vi "GDSLvIcon_GenerateObjectIcon.vi"(1 "HeaderColor":u32(colorbox)=786176, 3 "BackgroundColor":u32(colorbox)=16775072, 4 "Height":u32=22, 5 "error in (no error)":errorcluster, 6 "Type":T1, 7 "Width(30)":u32=30, 8 "ClassBodyIcon":string, 9 "_Thickness":u8=1 caption="Thickness (pixels)" min=1 max=3 step=1) -> (15 "BodyIconOut":u8[][](array[numeric])=[[2, 2, 2, 2, 2, 2, 2, 2, 2, 2, 2, 2, 2, 2, 2, 2, 2, 2, 2, 2, 2, 2, 2, 2, 2, 2, 2, 2, 2, 2], [2, 2, 2, 2, 2, 2, 2, 2, 2, 2, 2, 2, 2, 2, 185, 185, 2, 2, 2, 2, 2, 2, 2, 2, 2, 2, 2, 2, 2, 2], [2, 2, 2, 2, 2, 2, 2, 2, 2, 2, 2, 2, 185, 229, 227, 229, 229, 185, 2, 2, 2, 2, 2, 2, 2, 2, 2, 2, 2, 2], [2, 2, 2, 2, 2, 2, 2, 2, 2, 2, 185, 229, 227, 185, 185, 185, 185, 229, 229, 185, 2, 2, 2, 2, 2, 2, 2, 2, 2, 2], [2, 2, 2, 2, 2, 2, 2, 2, 185, 229, 227, 185, 185, 185, 185, 185, 185, 185, 185, 229, 229, 185, 2, 2, 2, 2, 2, 2, 2, 2], [2, 2, 2, 2, 2, 2, 2, 229, 227, 185, 185, 185, 185, 185, 185, 185, 185, 185, 185, 185, 185, 229, 229, 2, 2, 2, 2, 2, 2, 2], [2, 2, 2, 2, 2, 2, 2, 227, 227, 185, 185, 185, 185, 185, 185, 185, 185, 185, 185, 185, 185, 232, 229, 2, 2, 2, 2, 2, 2, 2], [2, 2, 2, 2, 2, 2, 2, 227, 229, 229, 227, 185, 185, 185, 185, 185, 185, 185, 185, 232, 232, 232, 227, 2, 2, 2, 2, 2, 2, 2], [2, 2, 2, 2, 2, 2, 2, 227, 229, 229, 229, 229, 227, 185, 185, 185, 185, 232, 232, 232, 232, 232, 227, 2, 2, 2, 2, 2, 2, 2], [2, 2, 2, 2, 2, 2, 2, 227, 229, 229, 229, 229, 229, 229, 227, 229, 232, 232, 232, 232, 232, 232, 227, 2, 2, 2, 2, 2, 2, 2], [2, 2, 2, 2, 2, 2, 2, 227, 229, 229, 229, 229, 229, 229, 229, 232, 232, 232, 232, 232, 232, 232, 227, 2, 2, 2, 2, 2, 2, 2], [2, 2, 2, 2, 2, 2, 2, 227, 229, 229, 229, 229, 229, 229, 229, 232, 232, 232, 232, 232, 232, 232, 227, 2, 2, 2, 2, 2, 2, 2], [2, 2, 2, 2, 2, 2, 2, 227, 229, 229, 229, 229, 229, 229, 229, 232, 232, 232, 232, 232, 232, 232, 227, 2, 2, 2, 2, 2, 2, 2], [2, 2, 2, 2, 2, 2, 2, 227, 229, 229, 229, 229, 229, 229, 229, 232, 232, 232, 232, 232, 232, 232, 227, 2, 2, 2, 2, 2, 2, 2], [2, 2, 2, 2, 2, 2, 2, 227, 229, 229, 229, 229, 229, 229, 229, 232, 232, 232, 232, 232, 232, 232, 227, 2, 2, 2, 2, 2, 2, 2], [2, 2, 2, 2, 2, 2, 2, 229, 229, 229, 229, 229, 229, 229, 229, 232, 232, 232, 232, 232, 232, 229, 229, 172, 172, 172, 2, 2, 2, 2], [2, 2, 2, 2, 2, 2, 2, 2, 227, 227, 229, 229, 229, 229, 229, 232, 232, 232, 232, 229, 229, 227, 172, 172, 172, 172, 172, 172, 2, 2], [2, 2, 2, 2, 2, 2, 2, 2, 2, 2, 227, 229, 229, 229, 229, 232, 232, 229, 229, 227, 172, 172, 172, 172, 172, 172, 2, 2, 2, 2], [2, 2, 2, 2, 2, 2, 2, 2, 2, 2, 2, 2, 227, 229, 229, 229, 229, 185, 172, 172, 172, 172, 172, 172, 172, 2, 2, 2, 2, 2], [2, 2, 2, 2, 2, 2, 2, 2, 2, 2, 2, 2, 2, 2, 227, 185, 172, 172, 172, 172, 172, 172, 172, 2, 2, 2, 2, 2, 2, 2], [2, 2, 2, 2, 2, 2, 2, 2, 2, 2, 2, 2, 2, 2, 2, 2, 2, 172, 172, 172, 172, 2, 2, 2, 2, 2, 2, 2, 2, 2], [2, 2, 2, 2, 2, 2, 2, 2, 2, 2, 2, 2, 2, 2, 2, 2, 2, 2, 2, 2, 2, 2, 2, 2, 2, 2, 2, 2, 2, 2]] format="%x", 19 "error out":errorcluster)   [LabVIEW 2020]
uses:
  <resource>/Framework/Providers/Open_GDS/ClassProviders/Common/LvIcon_class/GDSLvIcon_Type.ctl
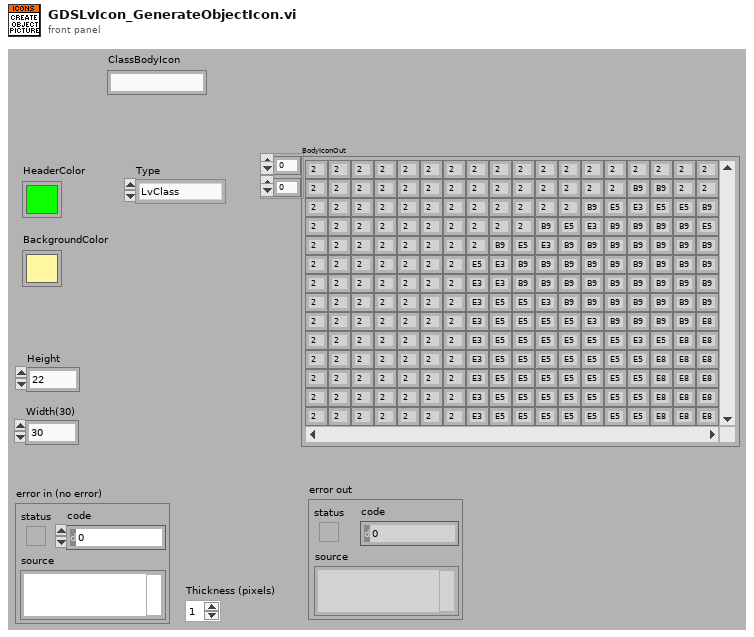
[diagram p1: front panel]
types:
  T1 = typedef "GDSLvIcon_Type.ctl" = enum16{"LvClass", "Library", "X-Control", "LvInterface"}
  T2 = typedef "imagedata.ctl" = cluster{"image type":i32, "image depth":i32, "image":u8[], "mask":u8[], "colors":u32[], "Rectangle":cluster{"left":i16, "top":i16, "right":i16, "bottom":i16}}
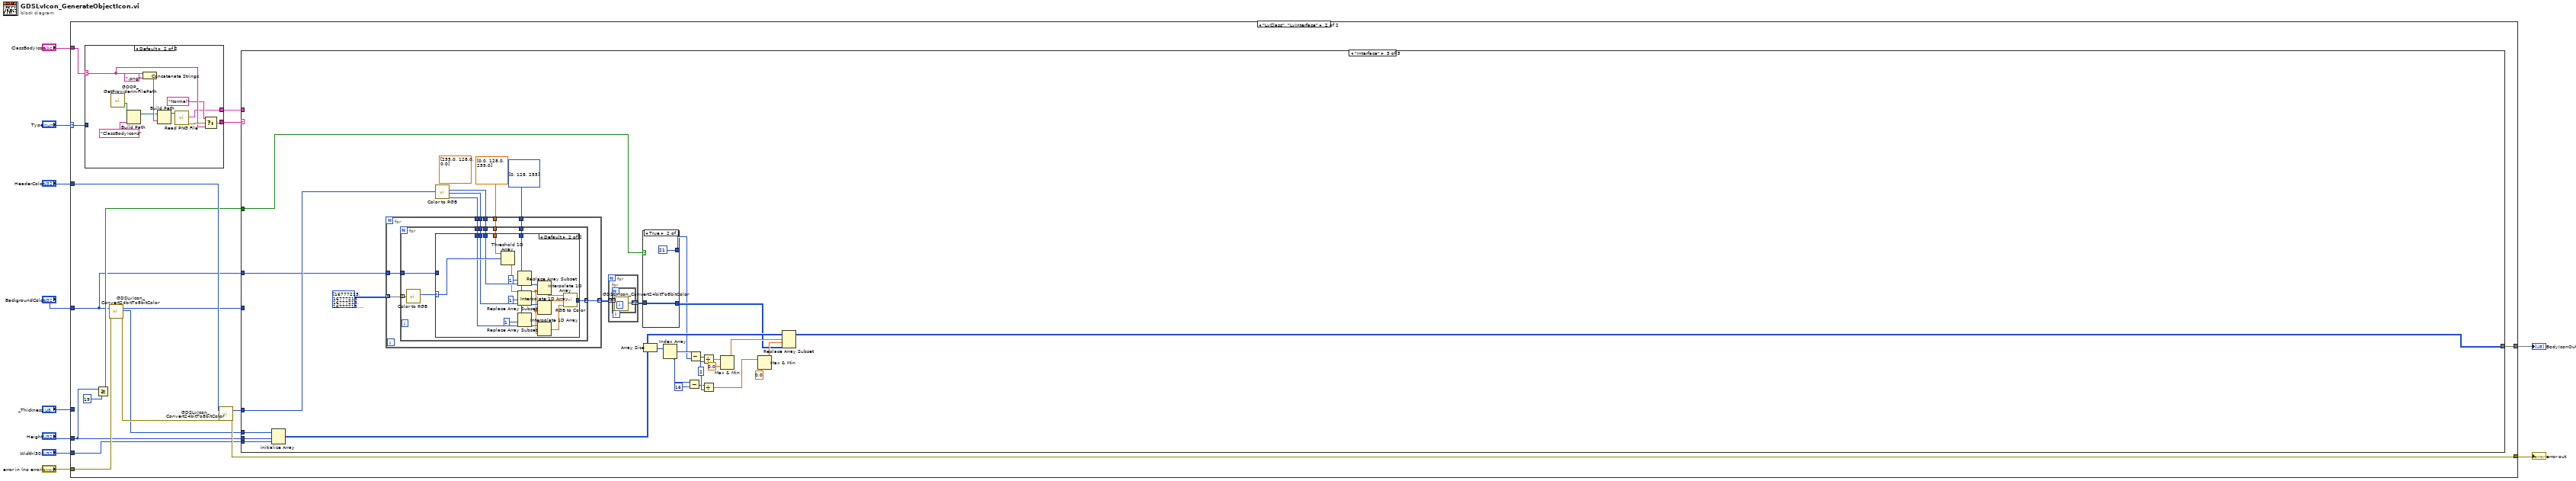
[diagram p0: block diagram]
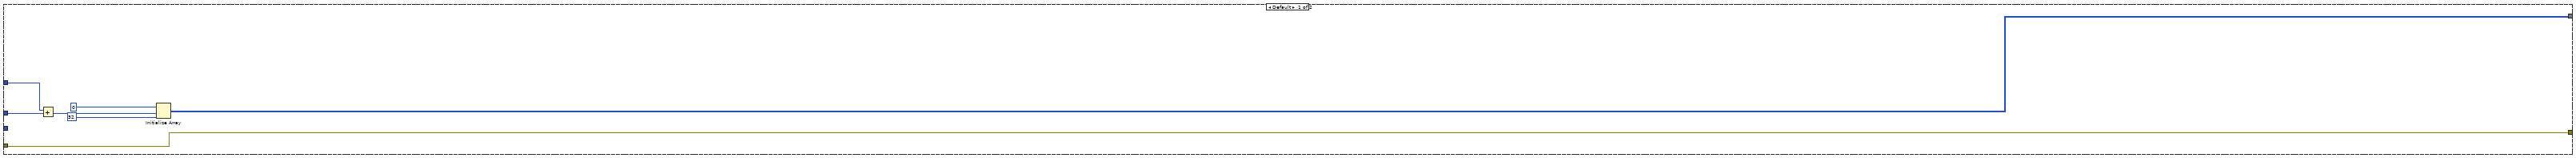
[diagram p2: hidden frame]
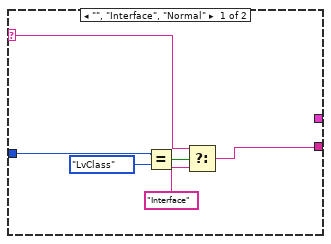
[diagram p3: hidden frame]
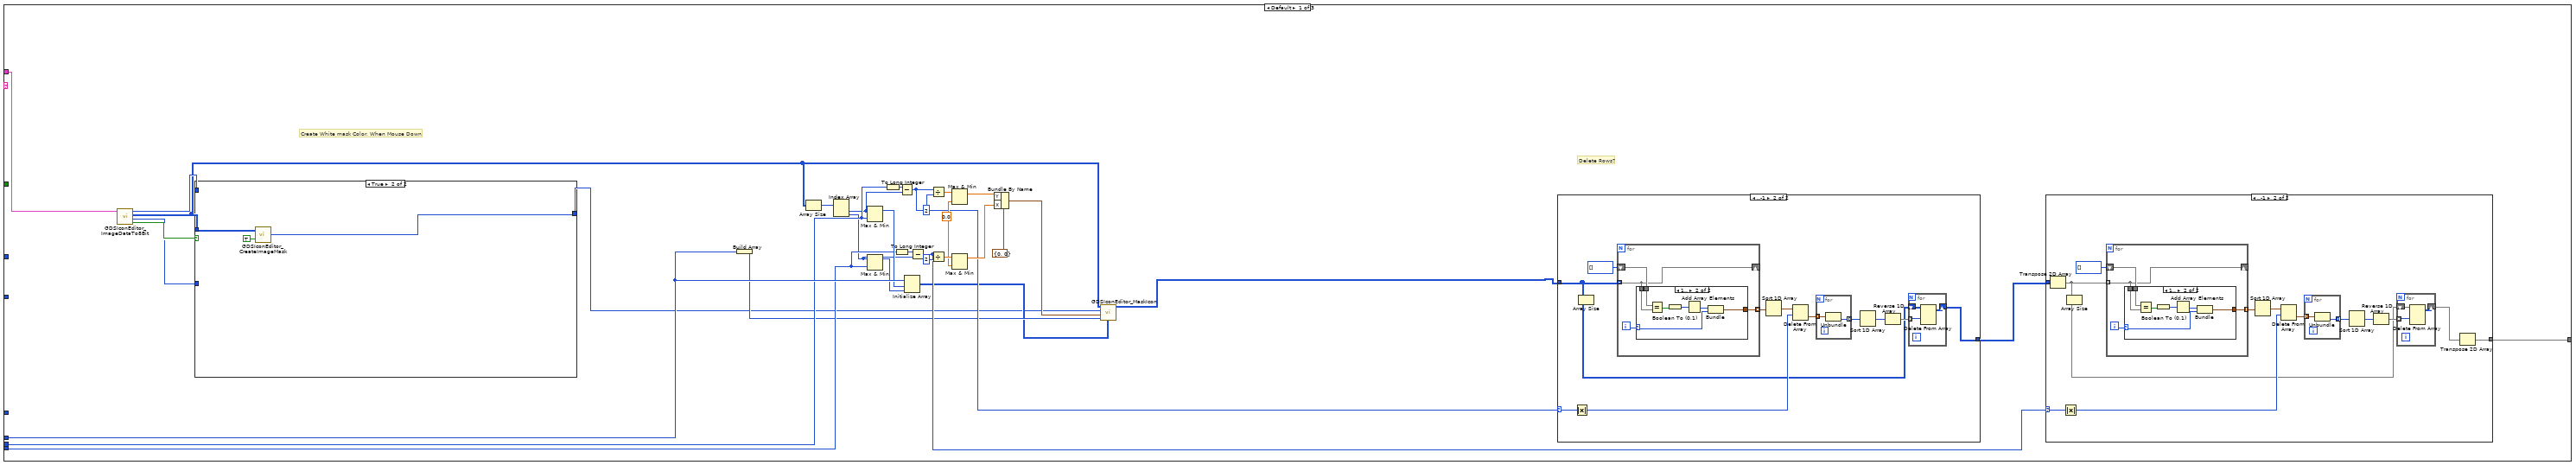
[diagram p4: hidden frame]
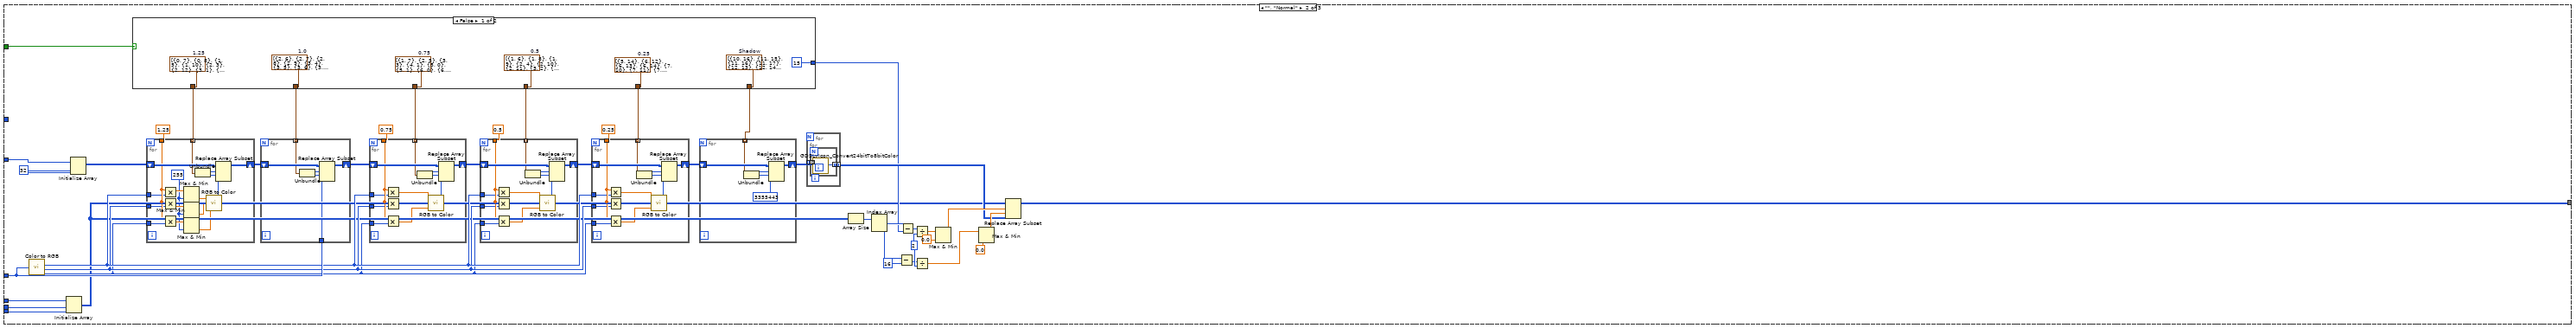
[diagram p10: hidden frame]
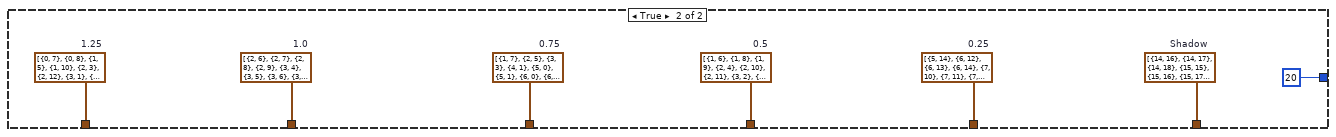
[diagram p11: hidden frame]
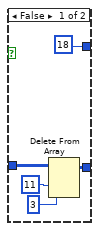
[diagram p12: hidden frame]
diagram:
  n1 = case shown="\"LvClass\", \"LvInterface\"" "Type" {
    selector: "Type" -> [_ w19]
    tunnel: "HeaderColor" -> [_ w34]
    tunnel: [w15 w32] -> w9
    tunnel: "BackgroundColor" -> [_ w18]
    tunnel: "error in (no error)" -> [w15 w31]
    tunnel: "Width(30)" -> [_ w20]
    tunnel: "Height" -> [w13 w21]
    tunnel: [w16 w24] -> w4
    tunnel: "_Thickness" -> [w12 _]
    tunnel: "ClassBodyIcon" -> [_ w26]
    frame Default {
      n2 = Add(x=w12, y=w13) -> (x+y=w11:u32)
      n3 = Initialize Array(u8 0 ("element"), w11, 32 ("dimension size")) -> (w16:u8[][])
    }
    frame "LvClass", "LvInterface" {
      n4 = case shown="Default" w26 {
        selector: w26 -> [w37 w44]
        tunnel: [w36 w43] -> w25
        tunnel: [_ w41] -> w23
        tunnel: w19 -> [w40 _]
        frame "", "Interface", "Normal" {
          n5 = Equal?(x=w40, y=GDSLvIcon_Type."LvClass") -> (x = y?=w38:bool)
          n6 = Select(t=w37, s=w38, f="Interface") -> (s? t:f=w36:string)
        }
        frame Default {
          n7 = call <resource>:"GOOP_GetProviderIniFilePath.vi"() -> ("ProviderMainFolder"=w48:path)  [unwired: 10 in, 1 out]
          n8 = Build Path(base path=w48, name or relative path="ClassBodyIcons") -> (appended path=w50:path)
          n9 = Concatenate Strings(w44, ".png" ("string")) -> (w51:string)
          n10 = Build Path(base path=w50, name or relative path=w51) -> (appended path=w46:path)
          n11 = call <vilib>:"Read PNG File.vi"("path to PNG file"=w46) -> ("error out"=w45:errorcluster, "image data"=w41:T2)  [unwired: 8 in, 1 out]
          n12 = Select(t="Normal", s=w45, f=w44) -> (s? t:f=w43:string)
        }
      }
      n13 = Greater Or Equal?(x=w21, y=19) -> (x >= y?=w28:bool)
      n14 = call <resource>:"GDSLvIcon_Convert24bitTo8bitColor.vi"("Color 24bit In"=w18, "error in (no error)"=w31) -> ("Adjusted 24bit Color Out"=w27:u32, "Color out(256)"=w22:u8, "error out"=w30:errorcluster)  [unwired: 14 in, 1 out]
      n15 = call <resource>:"GDSLvIcon_Convert24bitTo8bitColor.vi"("Color 24bit In"=w34, "error in (no error)"=w30) -> ("Adjusted 24bit Color Out"=w33:u32, "error out"=w32:errorcluster)  [unwired: 14 in, 2 out]
      n16 = case shown="\"Interface\"" w25 {
        tunnel: w33 -> [_ w186 w301]
        tunnel: w28 -> [_ w168 w277]
        tunnel: w27 -> [_ w167 _]
        tunnel: [w59 w150 w283] -> w24
        tunnel: w23 -> [w81 _ _]
        tunnel: w22 -> [w79 w149 w287]
        tunnel: w21 -> [w76 w148 w286]
        tunnel: w20 -> [w68 w147 w285]
        tunnel: w18 -> [_ _ w281]
        frame Default {
          w65 = 0.0 ("y")
          # "Delete Rows?"
          # "Create White mask Color, When Mouse Down"
          n17 = call <resource>:"GDSIconEditor_ImageDataTo8Bit.vi"("image data"=w81) -> ("NoMaskFound"=w83:bool, "ColorArray"=w58:u32[], "8-bit pixmap"=w55:u8[][], "mask"=w82:u8[])  [unwired: 7 in]
          n18 = case shown="True" w83 {
            tunnel: w55 -> [_ w145]
            tunnel: w82 -> [w142 _]
            tunnel: [w142 w143] -> w52
            tunnel: w58 -> [_ _]
            frame False {
            }
            frame True {
              n19 = call <resource>:"GDSIconEditor_CreateImageMask.vi"("Flood Fill"=TRUE, "8-bit pixmap"=w145) -> ("Array"=w143:u8[])
            }
          }
          n20 = Build Array(w79) -> (w56:u8[])
          n21 = Array Size(array=w55) -> (size(s)=w80:i32[])
          n22 = Index Array(array=w80) -> (element #1=w75:i32, element #2=w67:i32)  [unwired: 2 in]
          n23 = Max & Min(x=w75, y=w76) -> (max(x,y)=w78:u32)  [unwired: 1 out]
          n24 = Max & Min(x=w67, y=w68) -> (max(x,y)=w77:u32)  [unwired: 1 out]
          n25 = To Long Integer(number=w76) -> (32bit integer=w64:i32)
          n26 = To Long Integer(number=w68) -> (32bit integer=w63:i32)
          n27 = Subtract(x=w64, y=w75) -> (x-y=w62:i32)
          n28 = Initialize Array(w79, w78, w77) -> (w53:u8[][])
          n29 = Subtract(x=w63, y=w67) -> (x-y=w60:i32)
          n30 = Divide(x=w62, y=u32 2) -> (x/y=w73:dbl)
          n31 = Divide(x=w60, y=u32 2) -> (x/y=w70:dbl)
          n32 = Max & Min(x=w73, y=w65) -> (max(x,y)=w71:dbl)  [unwired: 1 out]
          n33 = Max & Min(x=w70, y=w65) -> (max(x,y)=w66:dbl)  [unwired: 1 out]
          n34 = Bundle By Name(cluster=cluster{"X":i32, "Y":i32} {"X"=0, "Y"=0} ("BgIconOffset"), "Y"=w71, "X"=w66) -> (w57:cluster{"X":i32, "Y":i32})
          n35 = call <resource>:"GDSIconEditor_MaskIcon.vi"("BgIcon"=w53, "ColorsOkayforiconToBeOnTopOf"=w56, "BgIconOffset"=w57, "BgIconMask"=w52, "IconIn"=w55) -> ("IconOut"=w54:u8[][])  [unwired: 6 in]
          n36 = case shown="..-1" w62 {
            selector: w62 -> [_ w125]
            tunnel: w54 -> [w114 w115]
            tunnel: [w114 w116] -> w61
            frame Default {
            }
            frame ..-1 {
              n37 = Absolute Value(x=w125) -> (abs(x)=w121:i32)
              n38 = Array Size(array=w115) -> ()  [unwired: 1 out]
              n39 = for {
                tunnel: w115 -> [w132] mode=indexing
                shift-right: [w132] -> _
                shift-left: u8[] [] -> [w133]
                tunnel: [w131] -> w123 mode=indexing
                i -> [w134]
                n40 = case shown="1.." w134 {
                  selector: w134 -> [_ w136]
                  tunnel: w133 -> [_ w141]
                  tunnel: w132 -> [_ w140]
                  tunnel: [_ w135] -> w131
                  frame 0, Default {
                  }
                  frame 1.. {
                    n41 = Equal?(x=w141, y=w140) -> (x = y?=w139:bool[])
                    n42 = Boolean To (0,1)(Boolean=w139) -> (0, 1=w138:i16[])
                    n43 = Add Array Elements(numeric array=w138) -> (sum=w137:i16)
                    n44 = Bundle("Color out(256)"=w137, w136) -> (w135:cluster{"Color out(256)":i16, i32})  [unwired: 1 in]
                  }
                }
              }
              n45 = Sort 1D Array(array=w123) -> (sorted array=w122:cluster{"Color out(256)":i16, i32}[])
              n46 = Delete From Array(array=w122, length=w121) -> (deleted portion=w120:cluster{"Color out(256)":i16, i32}[])  [unwired: 1 in, 1 out]
              n47 = for {
                tunnel: w120 -> [w130] mode=indexing
                tunnel: [w129] -> w119 mode=indexing
                n48 = Unbundle(w130) -> (w129:i32)  [unwired: 1 out]
              }
              n49 = Sort 1D Array(array=w119) -> (sorted array=w118:i32[])
              n50 = Reverse 1D Array(array=w118) -> (reversed array=w117:i32[])
              n51 = for {
                tunnel: w117 -> [w126] mode=indexing
                shift-right: [w127] -> w116
                shift-left: w115 -> [w128]
                n52 = Delete From Array(array=w128, index (row)=w126) -> (array with subset deleted=w127:u8[][])  [unwired: 2 in, 1 out]
              }
            }
          }
          n53 = case shown="..-1" w60 {
            selector: w60 -> [_ w97]
            tunnel: w61 -> [w84 w87]
            tunnel: [w84 w85] -> w59
            frame Default {
            }
            frame ..-1 {
              n54 = Transpose 2D Array(2D array=w87) -> (transposed array=w86:u8[][])
              n55 = Absolute Value(x=w97) -> (abs(x)=w93:i32)
              n56 = Array Size(array=w86) -> ()  [unwired: 1 out]
              n57 = for {
                tunnel: w86 -> [w104] mode=indexing
                shift-right: [w104] -> _
                shift-left: u8[] [] -> [w105]
                tunnel: [w103] -> w95 mode=indexing
                i -> [w106]
                n58 = case shown="1.." w106 {
                  selector: w106 -> [_ w108]
                  tunnel: w105 -> [_ w113]
                  tunnel: w104 -> [_ w112]
                  tunnel: [_ w107] -> w103
                  frame 0, Default {
                  }
                  frame 1.. {
                    n59 = Equal?(x=w113, y=w112) -> (x = y?=w111:bool[])
                    n60 = Boolean To (0,1)(Boolean=w111) -> (0, 1=w110:i16[])
                    n61 = Add Array Elements(numeric array=w110) -> (sum=w109:i16)
                    n62 = Bundle("Color out(256)"=w109, w108) -> (w107:cluster{"Color out(256)":i16, i32})  [unwired: 1 in]
                  }
                }
              }
              n63 = Sort 1D Array(array=w95) -> (sorted array=w94:cluster{"Color out(256)":i16, i32}[])
              n64 = Delete From Array(array=w94, length=w93) -> (deleted portion=w92:cluster{"Color out(256)":i16, i32}[])  [unwired: 1 in, 1 out]
              n65 = for {
                tunnel: w92 -> [w102] mode=indexing
                tunnel: [w101] -> w91 mode=indexing
                n66 = Unbundle(w102) -> (w101:i32)  [unwired: 1 out]
              }
              n67 = Sort 1D Array(array=w91) -> (sorted array=w90:i32[])
              n68 = Reverse 1D Array(array=w90) -> (reversed array=w89:i32[])
              n69 = for {
                tunnel: w89 -> [w98] mode=indexing
                shift-right: [w99] -> w88
                shift-left: w86 -> [w100]
                n70 = Delete From Array(array=w100, index (row)=w98) -> (array with subset deleted=w99:u8[][])  [unwired: 2 in, 1 out]
              }
              n71 = Transpose 2D Array(2D array=w88) -> (transposed array=w85:u8[][])
            }
          }
        }
        frame "", "Normal" {
          w157 = 2 ("y")
          w175 = 32 ("dimension size")
          n72 = call <vilib>:"Color to RGB.vi"("Color"=w186) -> ("R"=w178:u8, "G"=w177:u8, "B"=w176:u8)  [unwired: 1 out]
          n73 = Initialize Array(w149, w148, w147) -> (w146:u8[][])
          n74 = Initialize Array(w167, w175, w175) -> (w189:u32[][])
          n75 = case shown="False" w168 {
            tunnel: [w195 w207] -> w174
            tunnel: [w196 w206] -> w173
            tunnel: [w197 w205] -> w172
            tunnel: [w198 w204] -> w171
            tunnel: [w199 w203] -> w170
            tunnel: [w200 w202] -> w169
            tunnel: [15 ("y") 20 ("y")] -> w151
            frame False {
              w195 = cluster{"X":i32, "Y":i32}[] [{"X"=0, "Y"=7}, {"X"=0, "Y"=8}, {"X"=1, "Y"=5}, {"X"=1, "Y"=10}, {"X"=2, "Y"=3}, {"X"=2, "Y"=12}, {"X"=3, "Y"=1}, {"X"=3, "Y"=14}]  # 1.25
              w196 = cluster{"X":i32, "Y":i32}[] [{"X"=2, "Y"=6}, {"X"=2, "Y"=7}, {"X"=2, "Y"=8}, {"X"=2, "Y"=9}, {"X"=3, "Y"=4}, {"X"=3, "Y"=5}, {"X"=3, "Y"=6}, {"X"=3, "Y"=7}, {"X"=3, "Y"=8}, {"X"=3, "Y"=9}, {"X"=3, "Y"=10}, {"X"=3, "Y"=11}, {"X"=4, "Y"=2}, {"X"=4, "Y"=3}, {"X"=4, "Y"=4}, {"X"=4, "Y"=5}, {"X"=4, "Y"=6}, {"X"=4, "Y"=7}, {"X"=4, "Y"=8}, {"X"=4, "Y"=9}, {"X"=4, "Y"=10}, {"X"=4, "Y"=11}, {"X"=4, "Y"=12}, {"X"=4, "Y"=13}, {"X"=5, "Y"=2}, {"X"=5, "Y"=3}, {"X"=5, "Y"=4}, {"X"=5, "Y"=5}, {"X"=5, "Y"=6}, {"X"=5, "Y"=7}, {"X"=5, "Y"=8}, {"X"=5, "Y"=9}, {"X"=5, "Y"=10}, {"X"=5, "Y"=11}, {"X"=5, "Y"=12}, {"X"=5, "Y"=13}, {"X"=6, "Y"=4}, {"X"=6, "Y"=5}, {"X"=6, "Y"=6}, {"X"=6, "Y"=7}, {"X"=6, "Y"=8}, {"X"=6, "Y"=9}, {"X"=6, "Y"=10}, {"X"=6, "Y"=11}, {"X"=7, "Y"=6}, {"X"=7, "Y"=7}, {"X"=7, "Y"=8}, {"X"=7, "Y"=9}, {"X"=13, "Y"=10}, {"X"=14, "Y"=8}]  # 1.0
              w198 = cluster{"X":i32, "Y":i32}[] [{"X"=1, "Y"=6}, {"X"=1, "Y"=8}, {"X"=1, "Y"=9}, {"X"=2, "Y"=4}, {"X"=2, "Y"=10}, {"X"=2, "Y"=11}, {"X"=3, "Y"=2}, {"X"=3, "Y"=12}, {"X"=3, "Y"=13}, {"X"=4, "Y"=0}, {"X"=4, "Y"=14}, {"X"=4, "Y"=15}, {"X"=5, "Y"=15}, {"X"=6, "Y"=1}, {"X"=6, "Y"=2}, {"X"=7, "Y"=1}, {"X"=7, "Y"=2}, {"X"=7, "Y"=3}, {"X"=7, "Y"=4}, {"X"=8, "Y"=1}, {"X"=8, "Y"=2}, {"X"=8, "Y"=3}, {"X"=8, "Y"=4}, {"X"=8, "Y"=5}, {"X"=8, "Y"=6}, {"X"=8, "Y"=8}, {"X"=9, "Y"=1}, {"X"=9, "Y"=2}, {"X"=9, "Y"=3}, {"X"=9, "Y"=4}, {"X"=9, "Y"=5}, {"X"=9, "Y"=6}, {"X"=9, "Y"=7}, {"X"=10, "Y"=0}, {"X"=10, "Y"=1}, {"X"=10, "Y"=2}, {"X"=10, "Y"=3}, {"X"=10, "Y"=4}, {"X"=10, "Y"=5}, {"X"=10, "Y"=6}, {"X"=10, "Y"=7}, {"X"=10, "Y"=14}, {"X"=10, "Y"=15}, {"X"=11, "Y"=3}, {"X"=11, "Y"=4}, {"X"=11, "Y"=5}, {"X"=11, "Y"=6}, {"X"=11, "Y"=7}, {"X"=11, "Y"=12}, {"X"=11, "Y"=13}, {"X"=12, "Y"=4}, {"X"=12, "Y"=5}, {"X"=12, "Y"=6}, {"X"=12, "Y"=7}, {"X"=12, "Y"=10}, {"X"=12, "Y"=11}, {"X"=13, "Y"=6}, {"X"=13, "Y"=7}, {"X"=13, "Y"=8}, {"X"=13, "Y"=9}]  # 0.5
              w197 = cluster{"X":i32, "Y":i32}[] [{"X"=1, "Y"=7}, {"X"=2, "Y"=5}, {"X"=3, "Y"=3}, {"X"=4, "Y"=1}, {"X"=5, "Y"=0}, {"X"=5, "Y"=1}, {"X"=6, "Y"=0}, {"X"=6, "Y"=3}, {"X"=6, "Y"=15}, {"X"=7, "Y"=0}, {"X"=7, "Y"=5}, {"X"=7, "Y"=15}, {"X"=8, "Y"=0}, {"X"=8, "Y"=7}, {"X"=8, "Y"=15}, {"X"=9, "Y"=0}, {"X"=9, "Y"=15}, {"X"=11, "Y"=1}, {"X"=11, "Y"=2}, {"X"=11, "Y"=14}, {"X"=12, "Y"=3}, {"X"=12, "Y"=12}, {"X"=13, "Y"=5}, {"X"=14, "Y"=7}]  # 0.75
              w199 = cluster{"X":i32, "Y":i32}[] [{"X"=5, "Y"=14}, {"X"=6, "Y"=12}, {"X"=6, "Y"=13}, {"X"=6, "Y"=14}, {"X"=7, "Y"=10}, {"X"=7, "Y"=11}, {"X"=7, "Y"=12}, {"X"=7, "Y"=13}, {"X"=7, "Y"=14}, {"X"=8, "Y"=9}, {"X"=8, "Y"=10}, {"X"=8, "Y"=11}, {"X"=8, "Y"=12}, {"X"=8, "Y"=13}, {"X"=8, "Y"=14}, {"X"=9, "Y"=8}, {"X"=9, "Y"=9}, {"X"=9, "Y"=10}, {"X"=9, "Y"=11}, {"X"=9, "Y"=12}, {"X"=9, "Y"=13}, {"X"=9, "Y"=14}, {"X"=10, "Y"=8}, {"X"=10, "Y"=9}, {"X"=10, "Y"=10}, {"X"=10, "Y"=11}, {"X"=10, "Y"=12}, {"X"=10, "Y"=13}, {"X"=11, "Y"=8}, {"X"=11, "Y"=9}, {"X"=11, "Y"=10}, {"X"=11, "Y"=11}, {"X"=12, "Y"=8}, {"X"=12, "Y"=9}]  # 0.25
              w200 = cluster{"X":i32, "Y":i32}[] [{"X"=10, "Y"=16}, {"X"=11, "Y"=15}, {"X"=11, "Y"=16}, {"X"=11, "Y"=17}, {"X"=12, "Y"=13}, {"X"=12, "Y"=14}, {"X"=12, "Y"=15}, {"X"=12, "Y"=16}, {"X"=12, "Y"=17}, {"X"=13, "Y"=11}, {"X"=13, "Y"=12}, {"X"=13, "Y"=13}, {"X"=13, "Y"=14}, {"X"=13, "Y"=15}, {"X"=13, "Y"=16}, {"X"=14, "Y"=9}, {"X"=14, "Y"=10}, {"X"=14, "Y"=11}, {"X"=14, "Y"=12}, {"X"=14, "Y"=13}, {"X"=14, "Y"=14}, {"X"=14, "Y"=15}, {"X"=15, "Y"=10}, {"X"=15, "Y"=11}, {"X"=15, "Y"=12}, {"X"=15, "Y"=13}]  # Shadow
            }
            frame True {
              w202 = cluster{"X":i32, "Y":i32}[] [{"X"=14, "Y"=16}, {"X"=14, "Y"=17}, {"X"=14, "Y"=18}, {"X"=15, "Y"=15}, {"X"=15, "Y"=16}, {"X"=15, "Y"=17}, {"X"=15, "Y"=18}, {"X"=15, "Y"=19}, {"X"=15, "Y"=20}, {"X"=16, "Y"=13}, {"X"=16, "Y"=14}, {"X"=16, "Y"=15}, {"X"=16, "Y"=16}, {"X"=16, "Y"=17}, {"X"=16, "Y"=18}, {"X"=17, "Y"=11}, {"X"=17, "Y"=12}, {"X"=17, "Y"=13}, {"X"=17, "Y"=14}, {"X"=17, "Y"=15}, {"X"=17, "Y"=16}, {"X"=17, "Y"=17}, {"X"=18, "Y"=9}, {"X"=18, "Y"=10}, {"X"=18, "Y"=11}, {"X"=18, "Y"=12}, {"X"=18, "Y"=13}, {"X"=18, "Y"=14}, {"X"=18, "Y"=15}, {"X"=19, "Y"=10}, {"X"=19, "Y"=11}, {"X"=19, "Y"=12}, {"X"=19, "Y"=13}]  # Shadow
              w203 = cluster{"X":i32, "Y":i32}[] [{"X"=5, "Y"=14}, {"X"=6, "Y"=12}, {"X"=6, "Y"=13}, {"X"=6, "Y"=14}, {"X"=7, "Y"=10}, {"X"=7, "Y"=11}, {"X"=7, "Y"=12}, {"X"=7, "Y"=13}, {"X"=7, "Y"=14}, {"X"=8, "Y"=9}, {"X"=8, "Y"=10}, {"X"=8, "Y"=11}, {"X"=8, "Y"=12}, {"X"=8, "Y"=13}, {"X"=8, "Y"=14}, {"X"=9, "Y"=8}, {"X"=9, "Y"=9}, {"X"=9, "Y"=10}, {"X"=9, "Y"=11}, {"X"=9, "Y"=12}, {"X"=9, "Y"=13}, {"X"=9, "Y"=14}, {"X"=10, "Y"=8}, {"X"=10, "Y"=9}, {"X"=10, "Y"=10}, {"X"=10, "Y"=11}, {"X"=10, "Y"=12}, {"X"=10, "Y"=13}, {"X"=10, "Y"=14}, {"X"=11, "Y"=8}, {"X"=11, "Y"=9}, {"X"=11, "Y"=10}, {"X"=11, "Y"=11}, {"X"=11, "Y"=12}, {"X"=11, "Y"=13}, {"X"=11, "Y"=14}, {"X"=12, "Y"=8}, {"X"=12, "Y"=9}, {"X"=12, "Y"=10}, {"X"=12, "Y"=11}, {"X"=12, "Y"=12}, {"X"=12, "Y"=13}, {"X"=12, "Y"=14}, {"X"=13, "Y"=8}, {"X"=13, "Y"=9}, {"X"=13, "Y"=10}, {"X"=13, "Y"=11}, {"X"=13, "Y"=12}, {"X"=13, "Y"=13}, {"X"=13, "Y"=14}, {"X"=14, "Y"=8}, {"X"=14, "Y"=9}, {"X"=14, "Y"=10}, {"X"=14, "Y"=11}, {"X"=14, "Y"=12}, {"X"=14, "Y"=13}, {"X"=15, "Y"=8}, {"X"=15, "Y"=9}, {"X"=15, "Y"=10}, {"X"=15, "Y"=11}, {"X"=16, "Y"=8}, {"X"=16, "Y"=9}]  # 0.25
              w205 = cluster{"X":i32, "Y":i32}[] [{"X"=1, "Y"=7}, {"X"=2, "Y"=5}, {"X"=3, "Y"=3}, {"X"=4, "Y"=1}, {"X"=5, "Y"=0}, {"X"=5, "Y"=1}, {"X"=6, "Y"=0}, {"X"=6, "Y"=3}, {"X"=6, "Y"=15}, {"X"=7, "Y"=0}, {"X"=7, "Y"=5}, {"X"=7, "Y"=15}, {"X"=8, "Y"=0}, {"X"=8, "Y"=7}, {"X"=8, "Y"=15}, {"X"=9, "Y"=0}, {"X"=9, "Y"=15}, {"X"=10, "Y"=0}, {"X"=10, "Y"=15}, {"X"=11, "Y"=0}, {"X"=11, "Y"=15}, {"X"=12, "Y"=0}, {"X"=12, "Y"=15}, {"X"=13, "Y"=0}, {"X"=13, "Y"=15}, {"X"=15, "Y"=1}, {"X"=15, "Y"=2}, {"X"=15, "Y"=14}, {"X"=16, "Y"=3}, {"X"=16, "Y"=12}, {"X"=17, "Y"=5}, {"X"=18, "Y"=7}]  # 0.75
              w204 = cluster{"X":i32, "Y":i32}[] [{"X"=1, "Y"=6}, {"X"=1, "Y"=8}, {"X"=1, "Y"=9}, {"X"=2, "Y"=4}, {"X"=2, "Y"=10}, {"X"=2, "Y"=11}, {"X"=3, "Y"=2}, {"X"=3, "Y"=12}, {"X"=3, "Y"=13}, {"X"=4, "Y"=0}, {"X"=4, "Y"=14}, {"X"=4, "Y"=15}, {"X"=5, "Y"=15}, {"X"=6, "Y"=1}, {"X"=6, "Y"=2}, {"X"=7, "Y"=1}, {"X"=7, "Y"=2}, {"X"=7, "Y"=3}, {"X"=7, "Y"=4}, {"X"=8, "Y"=1}, {"X"=8, "Y"=2}, {"X"=8, "Y"=3}, {"X"=8, "Y"=4}, {"X"=8, "Y"=5}, {"X"=8, "Y"=6}, {"X"=8, "Y"=8}, {"X"=9, "Y"=1}, {"X"=9, "Y"=2}, {"X"=9, "Y"=3}, {"X"=9, "Y"=4}, {"X"=9, "Y"=5}, {"X"=9, "Y"=6}, {"X"=9, "Y"=7}, {"X"=10, "Y"=1}, {"X"=10, "Y"=2}, {"X"=10, "Y"=3}, {"X"=10, "Y"=4}, {"X"=10, "Y"=5}, {"X"=10, "Y"=6}, {"X"=10, "Y"=7}, {"X"=11, "Y"=1}, {"X"=11, "Y"=2}, {"X"=11, "Y"=3}, {"X"=11, "Y"=4}, {"X"=11, "Y"=5}, {"X"=11, "Y"=6}, {"X"=11, "Y"=7}, {"X"=12, "Y"=1}, {"X"=12, "Y"=2}, {"X"=12, "Y"=3}, {"X"=12, "Y"=4}, {"X"=12, "Y"=5}, {"X"=12, "Y"=6}, {"X"=12, "Y"=7}, {"X"=13, "Y"=1}, {"X"=13, "Y"=2}, {"X"=13, "Y"=3}, {"X"=13, "Y"=4}, {"X"=13, "Y"=5}, {"X"=13, "Y"=6}, {"X"=13, "Y"=7}, {"X"=14, "Y"=0}, {"X"=14, "Y"=1}, {"X"=14, "Y"=2}, {"X"=14, "Y"=3}, {"X"=14, "Y"=4}, {"X"=14, "Y"=5}, {"X"=14, "Y"=6}, {"X"=14, "Y"=7}, {"X"=14, "Y"=14}, {"X"=14, "Y"=15}, {"X"=15, "Y"=3}, {"X"=15, "Y"=4}, {"X"=15, "Y"=5}, {"X"=15, "Y"=6}, {"X"=15, "Y"=7}, {"X"=15, "Y"=12}, {"X"=15, "Y"=13}, {"X"=16, "Y"=4}, {"X"=16, "Y"=5}, {"X"=16, "Y"=6}, {"X"=16, "Y"=7}, {"X"=16, "Y"=10}, {"X"=16, "Y"=11}, {"X"=17, "Y"=6}, {"X"=17, "Y"=7}, {"X"=17, "Y"=8}, {"X"=17, "Y"=9}]  # 0.5
              w206 = cluster{"X":i32, "Y":i32}[] [{"X"=2, "Y"=6}, {"X"=2, "Y"=7}, {"X"=2, "Y"=8}, {"X"=2, "Y"=9}, {"X"=3, "Y"=4}, {"X"=3, "Y"=5}, {"X"=3, "Y"=6}, {"X"=3, "Y"=7}, {"X"=3, "Y"=8}, {"X"=3, "Y"=9}, {"X"=3, "Y"=10}, {"X"=3, "Y"=11}, {"X"=4, "Y"=2}, {"X"=4, "Y"=3}, {"X"=4, "Y"=4}, {"X"=4, "Y"=5}, {"X"=4, "Y"=6}, {"X"=4, "Y"=7}, {"X"=4, "Y"=8}, {"X"=4, "Y"=9}, {"X"=4, "Y"=10}, {"X"=4, "Y"=11}, {"X"=4, "Y"=12}, {"X"=4, "Y"=13}, {"X"=5, "Y"=2}, {"X"=5, "Y"=3}, {"X"=5, "Y"=4}, {"X"=5, "Y"=5}, {"X"=5, "Y"=6}, {"X"=5, "Y"=7}, {"X"=5, "Y"=8}, {"X"=5, "Y"=9}, {"X"=5, "Y"=10}, {"X"=5, "Y"=11}, {"X"=5, "Y"=12}, {"X"=5, "Y"=13}, {"X"=6, "Y"=4}, {"X"=6, "Y"=5}, {"X"=6, "Y"=6}, {"X"=6, "Y"=7}, {"X"=6, "Y"=8}, {"X"=6, "Y"=9}, {"X"=6, "Y"=10}, {"X"=6, "Y"=11}, {"X"=7, "Y"=6}, {"X"=7, "Y"=7}, {"X"=7, "Y"=8}, {"X"=7, "Y"=9}, {"X"=17, "Y"=10}, {"X"=18, "Y"=8}]  # 1.0
              w207 = cluster{"X":i32, "Y":i32}[] [{"X"=0, "Y"=7}, {"X"=0, "Y"=8}, {"X"=1, "Y"=5}, {"X"=1, "Y"=10}, {"X"=2, "Y"=3}, {"X"=2, "Y"=12}, {"X"=3, "Y"=1}, {"X"=3, "Y"=14}]  # 1.25
            }
          }
          n76 = for {
            shift-right: [w274] -> w187
            shift-left: w189 -> [w275]
            tunnel: w174 -> [w260] mode=indexing
            tunnel: 1.25 ("upper limit") -> [w266]
            tunnel: w178 -> [w265]
            tunnel: w177 -> [w264]
            tunnel: w176 -> [w263]
            w267 = 255 ("upper limit")
            n77 = Multiply(x=w266, y=w265) -> (x*y=w273:dbl)
            n78 = Multiply(x=w266, y=w264) -> (x*y=w269:dbl)
            n79 = Multiply(x=w266, y=w263) -> (x*y=w268:dbl)
            n80 = Max & Min(x=w273, y=w267) -> (min(x,y)=w272:dbl)  [unwired: 1 out]
            n81 = Max & Min(x=w269, y=w267) -> (min(x,y)=w271:dbl)  [unwired: 1 out]
            n82 = Max & Min(x=w268, y=w267) -> (min(x,y)=w270:dbl)  [unwired: 1 out]
            n83 = Unbundle(w260) -> ("X"=w261:i32, "Y"=w259:i32)
            n84 = call <vilib>:"RGB to Color.vi"("B"=w270, "G"=w271, "R"=w272) -> ("Color"=w262:u32)
            n85 = Replace Array Subset(array=w275, new element=w262, index (row)=w261, index (col)=w259) -> (w274:u32[][])
          }
          n86 = for {
            shift-right: [w257] -> w184
            shift-left: w187 -> [w258]
            tunnel: w173 -> [w256] mode=indexing
            tunnel: w186 -> [w255]
            n87 = Unbundle(w256) -> ("X"=w254:i32, "Y"=w253:i32)
            n88 = Replace Array Subset(array=w258, new element=w255, index (row)=w254, index (col)=w253) -> (w257:u32[][])
          }
          n89 = for {
            shift-right: [w251] -> w182
            shift-left: w184 -> [w252]
            tunnel: w172 -> [w250] mode=indexing
            tunnel: 0.75 ("upper limit") -> [w249]
            tunnel: w178 -> [w248]
            tunnel: w177 -> [w247]
            tunnel: w176 -> [w246]
            n90 = Multiply(x=w249, y=w248) -> (x*y=w244:dbl)
            n91 = Multiply(x=w249, y=w247) -> (x*y=w243:dbl)
            n92 = Multiply(x=w249, y=w246) -> (x*y=w242:dbl)
            n93 = Unbundle(w250) -> ("X"=w241:i32, "Y"=w240:i32)
            n94 = call <vilib>:"RGB to Color.vi"("B"=w242, "G"=w243, "R"=w244) -> ("Color"=w245:u32)
            n95 = Replace Array Subset(array=w252, new element=w245, index (row)=w241, index (col)=w240) -> (w251:u32[][])
          }
          n96 = for {
            shift-right: [w238] -> w180
            shift-left: w182 -> [w239]
            tunnel: w171 -> [w237] mode=indexing
            tunnel: 0.5 ("upper limit") -> [w236]
            tunnel: w178 -> [w235]
            tunnel: w177 -> [w234]
            tunnel: w176 -> [w233]
            n97 = Multiply(x=w236, y=w235) -> (x*y=w231:dbl)
            n98 = Multiply(x=w236, y=w234) -> (x*y=w230:dbl)
            n99 = Multiply(x=w236, y=w233) -> (x*y=w229:dbl)
            n100 = Unbundle(w237) -> ("X"=w228:i32, "Y"=w227:i32)
            n101 = call <vilib>:"RGB to Color.vi"("B"=w229, "G"=w230, "R"=w231) -> ("Color"=w232:u32)
            n102 = Replace Array Subset(array=w239, new element=w232, index (row)=w228, index (col)=w227) -> (w238:u32[][])
          }
          n103 = for {
            shift-right: [w225] -> w179
            shift-left: w180 -> [w226]
            tunnel: w170 -> [w224] mode=indexing
            tunnel: 0.25 ("upper limit") -> [w223]
            tunnel: w178 -> [w222]
            tunnel: w177 -> [w221]
            tunnel: w176 -> [w220]
            n104 = Multiply(x=w223, y=w222) -> (x*y=w218:dbl)
            n105 = Multiply(x=w223, y=w221) -> (x*y=w217:dbl)
            n106 = Multiply(x=w223, y=w220) -> (x*y=w216:dbl)
            n107 = Unbundle(w224) -> ("X"=w215:i32, "Y"=w214:i32)
            n108 = call <vilib>:"RGB to Color.vi"("B"=w216, "G"=w217, "R"=w218) -> ("Color"=w219:u32)
            n109 = Replace Array Subset(array=w226, new element=w219, index (row)=w215, index (col)=w214) -> (w225:u32[][])
          }
          n110 = for {
            shift-right: [w212] -> w166
            shift-left: w179 -> [w213]
            tunnel: w169 -> [w211] mode=indexing
            n111 = Unbundle(w211) -> ("X"=w209:i32, "Y"=w208:i32)
            n112 = Replace Array Subset(array=w213, new element=u32 3355443 ("new element/subarray"), index (row)=w209, index (col)=w208) -> (w212:u32[][])
          }
          n113 = for {
            tunnel: w166 -> [w191] mode=indexing
            tunnel: [w190] -> w152 mode=indexing
            n114 = for {
              tunnel: w191 -> [w193] mode=indexing
              tunnel: [w192] -> w190 mode=indexing
              n115 = call <resource>:"GDSLvIcon_Convert24bitTo8bitColor.vi"("Color 24bit In"=w193) -> ("Color out(256)"=w192:u8)  [unwired: 15 in, 3 out]
            }
          }
          n116 = Array Size(array=w146) -> (size(s)=w153:i32[])
          n117 = Index Array(array=w153) -> (element #1=w154:i32, element #2=w158:i32)  [unwired: 2 in]
          n118 = Subtract(x=w158, y=16) -> (x-y=w156:i32)
          n119 = Subtract(x=w154, y=w151) -> (x-y=w155:i32)
          n120 = Divide(x=w155, y=w157) -> (x/y=w161:dbl)
          n121 = Divide(x=w156, y=w157) -> (x/y=w164:dbl)
          n122 = Max & Min(x=w161, y=0.0) -> (max(x,y)=w162:dbl)  [unwired: 1 out]
          n123 = Max & Min(x=w164, y=0.0) -> (max(x,y)=w165:dbl)  [unwired: 1 out]
          n124 = Replace Array Subset(array=w146, new element=w152, index (row)=w162, index (col)=w165) -> (w150:u8[][])
        }
        frame "Interface" {
          w292 = 2 ("y")
          (unwired) sgl[] [255.0, 128.0, 0.0]
          n125 = Initialize Array(w287, w286, w285) -> (w284:u8[][])
          n126 = call <vilib>:"Color to RGB.vi"("Color"=w301) -> ("R"=w304:u8, "G"=w305:u8, "B"=w306:u8)  [unwired: 1 out]
          n127 = for {
            tunnel: u32[][] [[16777215, 16777215, 16777215, 16777215, 16777215, 16777215, 16777215, 16777215, 10658466, 10658466, 16777215, 16777215, 16777215, 16777215, 16777215, 16777215, 16777215, 16777215], [16777215, 16777215, 16777215, 16777215, 16777215, 16777215, 10724259, 10724259, 10592673, 10592673, 10658466, 10658466, 16777215, 16777215, 16777215, 16777215, 16777215, 16777215], [16777215, 16777215, 16777215, 16777215, 12500670, 10658466, 10658466, 10592673, 10592673, 10592673, 10592673, 10592673, 10724259, 10724259, 16777215, 16777215, 16777215, 16777215], [16777215, 16777215, 16777215, 11842740, 10592673, 10592673, 10592673, 10592673, 10592673, 10592673, 10592673, 10592673, 10592673, 10658466, 10658466, 10724259, 16777215, 16777215], [16777215, 10855845, 10724259, 10592673, 10592673, 10592673, 10592673, 10592673, 10592673, 10592673, 10592673, 10592673, 10592673, 10592673, 10592673, 10592673, 13619151, 16777215], [16777215, 14342874, 10921638, 10592673, 10592673, 10592673, 10592673, 10592673, 10592673, 10592673, 10592673, 10592673, 10592673, 10592673, 10592673, 10724259, 15198183, 16777215], [10658466, 16711422, 16250871, 13948116, 10592673, 10592673, 10592673, 10592673, 10592673, 10592673, 10592673, 10592673, 10592673, 10790052, 13158600, 15658734, 16448250, 13553358], [6052956, 9013641, 15790320, 16711422, 13487565, 11250603, 10592673, 10592673, 10592673, 10592673, 10592673, 10592673, 11645361, 16053492, 16711422, 16119285, 3552822, 2105376], [6052956, 6316128, 6710886, 9671571, 16711422, 16514043, 14671839, 10592673, 10592673, 10592673, 12040119, 14474460, 16645629, 15592941, 7171437, 2894892, 1973790, 1973790], [6052956, 6316128, 6316128, 6316128, 10395294, 15198183, 16579836, 14342874, 12040119, 14079702, 16711422, 16711422, 12237498, 2434341, 1973790, 1973790, 1973790, 1973790], [6052956, 6316128, 6316128, 6316128, 6316128, 6513507, 8618883, 16645629, 16579836, 16711422, 10658466, 4408131, 2039583, 1973790, 1973790, 1973790, 1973790, 1973790], [6052956, 6316128, 6316128, 6316128, 6316128, 6316128, 6316128, 13421772, 16316664, 15856113, 2631720, 1973790, 1973790, 1973790, 1973790, 1973790, 1973790, 1973790], [6052956, 6316128, 6316128, 6316128, 6316128, 6316128, 6316128, 6974058, 14277081, 15198183, 1973790, 1973790, 1973790, 1973790, 1973790, 1973790, 1973790, 1973790], [6052956, 6316128, 6316128, 6316128, 6316128, 6316128, 6316128, 6974058, 14211288, 15132390, 1973790, 1973790, 1973790, 1973790, 1973790, 1973790, 1973790, 1973790], [5592405, 6316128, 6316128, 6316128, 6316128, 6316128, 6316128, 6974058, 14211288, 15132390, 1973790, 1973790, 1973790, 1973790, 1973790, 1973790, 1973790, 16777215], [16777215, 5987163, 6316128, 6316128, 6316128, 6316128, 6316128, 6974058, 14211288, 15132390, 1973790, 1973790, 1973790, 1973790, 1973790, 1973790, 5395026, 16777215], [16777215, 16777215, 10263708, 6118749, 6316128, 6316128, 6316128, 6974058, 14211288, 15132390, 1973790, 1973790, 1973790, 1973790, 2368548, 5460819, 16777215, 16777215], [16777215, 16777215, 16777215, 14606046, 6381921, 6250335, 6316128, 6974058, 14211288, 15132390, 1973790, 1973790, 1973790, 5395026, 6710886, 16777215, 16777215, 16777215], [16777215, 16777215, 16777215, 16777215, 16777215, 12369084, 9079434, 6974058, 14211288, 15132390, 1973790, 2763306, 5131854, 9671571, 16777215, 16777215, 16777215, 16777215], [16777215, 16777215, 16777215, 16777215, 16777215, 16777215, 16777215, 9934743, 14277081, 15132390, 5197647, 7171437, 11382189, 16777215, 16777215, 16777215, 16777215, 16777215], [16777215, 16777215, 16777215, 16777215, 16777215, 16777215, 16777215, 16777215, 16119285, 16119285, 11842740, 16777215, 16777215, 16777215, 16777215, 16777215, 16777215, 16777215]] ("24-bit pixmap") -> [w325] mode=indexing
            tunnel: [w324] -> w282 mode=indexing
            tunnel: w306 -> [w323]
            tunnel: w305 -> [w322]
            tunnel: w304 -> [w321]
            tunnel: sgl[] [0.0, 128.0, 255.0] -> [w320]
            tunnel: u8[] [0, 128, 255] -> [w319]
            tunnel: w281 -> [w318]
            n128 = for {
              tunnel: w325 -> [w334] mode=indexing
              tunnel: [w333] -> w324 mode=indexing
              tunnel: w323 -> [w327]
              tunnel: w322 -> [w328]
              tunnel: w321 -> [w330]
              tunnel: w320 -> [w332]
              tunnel: w319 -> [w329]
              tunnel: w318 -> [w326]
              n129 = call <vilib>:"Color to RGB.vi"("Color"=w334) -> ("R"=w331:u8)  [unwired: 3 out]
              n130 = case shown="Default" w331 {
                selector: w331 -> [_ w350]
                tunnel: [w335 w352] -> w333
                tunnel: w332 -> [_ w351]
                tunnel: w330 -> [_ w348]
                tunnel: w329 -> [_ w341]
                tunnel: w328 -> [_ w339]
                tunnel: w327 -> [_ w338]
                tunnel: w326 -> [w335 _]
                frame 255 {
                }
                frame Default {
                  n131 = Threshold 1D Array(2:w350, 3:w351) -> (0:w340:sgl)  [unwired: 1 in]
                  n132 = Replace Array Subset(array=w341, new element=w348, index=1) -> (w347:u8[])
                  n133 = Replace Array Subset(array=w341, new element=w339, index=1) -> (w345:u8[])
                  n134 = Replace Array Subset(array=w341, new element=w338, index=1) -> (w342:u8[])
                  n135 = Interpolate 1D Array(1:w340, 2:w347) -> (0:w346:dbl)
                  n136 = Interpolate 1D Array(1:w340, 2:w345) -> (0:w337:dbl)
                  n137 = Interpolate 1D Array(1:w340, 2:w342) -> (0:w336:dbl)
                  n138 = call <vilib>:"RGB to Color.vi"("B"=w336, "G"=w337, "R"=w346) -> ("Color"=w352:u32)
                }
              }
            }
          }
          n139 = for {
            tunnel: w282 -> [w315] mode=indexing
            tunnel: [w314] -> w279 mode=indexing
            n140 = for {
              tunnel: w315 -> [w317] mode=indexing
              tunnel: [w316] -> w314 mode=indexing
              n141 = call <resource>:"GDSLvIcon_Convert24bitTo8bitColor.vi"("Color 24bit In"=w317) -> ("Color out(256)"=w316:u8)  [unwired: 15 in, 3 out]
            }
          }
          n142 = case shown="True" w277 {
            tunnel: w279 -> [w309 w313]
            tunnel: [w308 w313] -> w278
            tunnel: [18 ("y") 21 ("y")] -> w276
            frame False {
              n143 = Delete From Array(array=w309, length=3, index (row)=11) -> (array with subset deleted=w308:u8[][])  [unwired: 1 in, 1 out]
            }
            frame True {
            }
          }
          n144 = Array Size(array=w284) -> (size(s)=w288:i32[])
          n145 = Index Array(array=w288) -> (element #1=w289:i32, element #2=w293:i32)  [unwired: 2 in]
          n146 = Subtract(x=w293, y=16) -> (x-y=w291:i32)
          n147 = Subtract(x=w289, y=w276) -> (x-y=w290:i32)
          n148 = Divide(x=w290, y=w292) -> (x/y=w296:dbl)
          n149 = Divide(x=w291, y=w292) -> (x/y=w299:dbl)
          n150 = Max & Min(x=w296, y=0.0) -> (max(x,y)=w297:dbl)  [unwired: 1 out]
          n151 = Max & Min(x=w299, y=0.0) -> (max(x,y)=w300:dbl)  [unwired: 1 out]
          n152 = Replace Array Subset(array=w284, new element=w278, index (row)=w297, index (col)=w300) -> (w283:u8[][])
        }
      }
    }
  }
  "error out" <- w9
  "BodyIconOut" <- w4
